vi "Close All Message Queues.vi"(8 "error in (no error)":errorcluster, 10 "force destroy? (F)":bool, 11 "Message Queues":T1) -> (0 "error out":errorcluster)   [LabVIEW 2026, in "Message Queue.lvlib"]
doc: "すべてのメッセージキューを破棄します。"
uses:
  Message Queue.lvlib
  All Message Queues.ctl
  Message Cluster.ctl
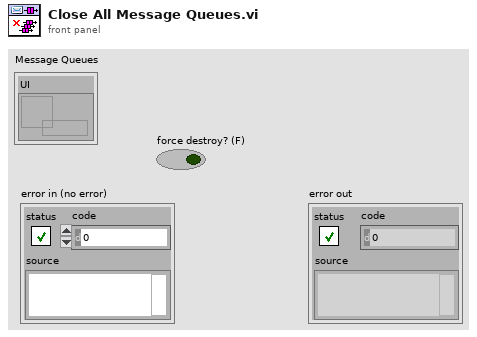
[diagram p1: front panel]
types:
  T1 = typedef "Message Queue.lvlib/All Message Queues.ctl" = cluster{"UI":refnum<queue>}
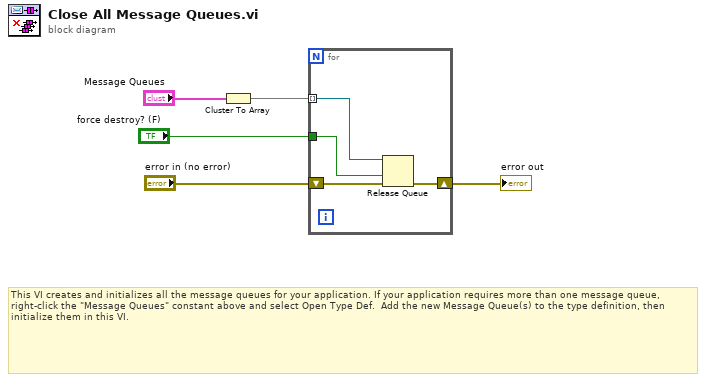
[diagram p0: block diagram]
diagram:
  # "This VI creates and initializes all the message queues for your application. If your application requires more than one message queue, right-click the \"Message Queues\" constant above and select Open Type Def.  Add the new Message Queue(s) to the type definition, then initialize them in this VI."
  n1 = Cluster To Array(cluster="Message Queues") -> (array=w2:refnum<queue>[])
  n2 = for {
    shift-right: [w8] -> w3
    shift-left: "error in (no error)" -> [w9]
    tunnel: w2 -> [w7] mode=indexing
    tunnel: "force destroy? (F)" -> [w6]
    n3 = Release Queue(queue=w7, force destroy? (F)=w6, error in (no error)=w9) -> (error out=w8:errorcluster)  [unwired: 2 out]
  }
  "error out" <- w3
